vi "layout.vi"(0 "reference in":refnum<class "DQMHModuleNode.lvclass">, 1 "graph":refnum<class "Graph.lvclass">, 2 "graphics":refnum<class "Graphics.lvclass">, 3 "grid":refnum<class "Grid.lvclass">, 5 "error in (no error)":errorcluster) -> (14 "reference out":refnum<class "DQMHModuleNode.lvclass">, 19 "error out":errorcluster)   [LabVIEW 2020, in "DQMHModuleNode.lvclass"]
doc: "public void layout(Graph g, Graphics2D g2, Grid grid)"
uses:
  <resource>/Framework/Providers/Open_GDS/UML/DQMHModuleNode_class/DQMHModuleNode.lvclass
  C:/Program Files (x86)/National Instruments/LabVIEW 2020/resource/Framework/Providers/Open_GDS/UML/RectangularNode_class/RectangularNode.lvclass
  <resource>/Framework/Providers/Open_GDS/UML/Graph_class/Graph.lvclass
  <resource>/Framework/Providers/Open_GDS/UML/Graphics_class/Graphics.lvclass
  <resource>/Framework/Providers/Open_GDS/UML/Grid_class/Grid.lvclass
  <resource>/Framework/Providers/Open_GDS/UML/MultiLineString_class/MultiLineString.lvclass
  <resource>/Framework/Providers/Open_GDS/UML/RectangularNode_class/RectangularNode.lvclass
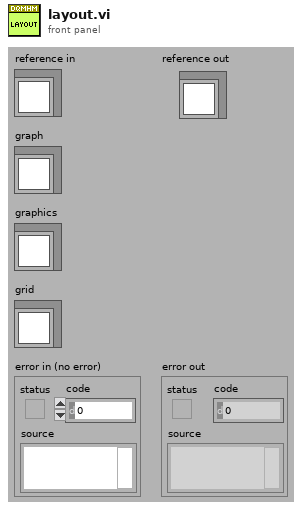
[diagram p1: front panel]
types:
  T1 = typedef "DQMHModuleNode.lvclass/ObjectAttributes.ctl" = cluster{"DescriptionHeight":dbl, "InternalDataHeight":dbl, "EventsHeight":dbl, "Name":refnum<class "MultiLineString.lvclass">, "Description":refnum<class "MultiLineString.lvclass">, "InternalData":refnum<class "MultiLineString.lvclass">, "Events":refnum<class "MultiLineString.lvclass">, "showDescription":bool, "showInternalData":bool, "showEvents":bool, "DEFAULT_ROUNDING":i32, "DEFAULT_WIDTH":i32, "DEFAULT_HEIGHT":i32, "ClassPath":path, "Template":string, "Icon":u8[][]}
  T2 = typedef "RectangularNode.lvclass/ObjectAttributes.ctl" = cluster{"bounds":T3}
  T3 = typedef "Rectangle Rectangle2D.ctl" = cluster{"x":dbl, "y":dbl, "width":dbl, "height":dbl}
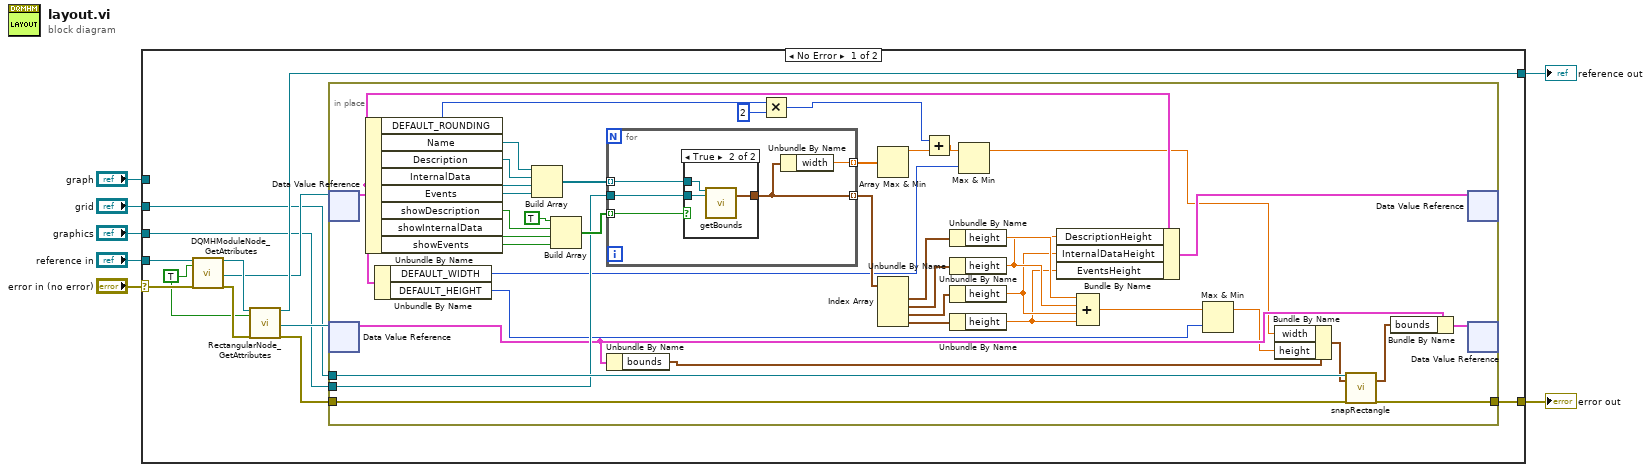
[diagram p0: block diagram]
diagram:
  n1 = case shown="No Error" "error in (no error)" {
    selector: "error in (no error)" -> [w16 w69]
    tunnel: "reference in" -> [w19 w70]
    tunnel: [w18 w69] -> w6
    tunnel: [w17 w70] -> w5
    tunnel: "graph" -> [_ _]
    tunnel: "graphics" -> [w10 _]
    tunnel: "grid" -> [w9 _]
    frame No Error {
      w8 = TRUE ("OnlyGetDvrReference(False)")
      n2 = call <resource>:"DQMHModuleNode_GetAttributes.vi"("reference in"=w19, "OnlyGetDvrReference(False)"=w8, "error in (no error)"=w16) -> ("reference out"=w15:refnum<class "DQMHModuleNode.lvclass">, "DataRef"=w13:refnum<data-value>, "error out"=w14:errorcluster)  [unwired: 13 in, 1 out]
      n3 = call <resource>:"RectangularNode_GetAttributes.vi"("reference in"=w15, "OnlyGetDvrReference(False)"=w8, "error in (no error)"=w14) -> ("reference out"=w17:refnum<class "DQMHModuleNode.lvclass">, "DataRef"=w12:refnum<data-value>, "error out"=w11:errorcluster)  [unwired: 13 in, 1 out]
      n4 = in-place {
        in-place-border: w11 -> [w25]
        in-place-border: w10 -> [w42]
        in-place-border: w9 -> [w59]
        in-place-border: [w57] -> w18
        n5 = in-place-dvr #1(w13) -> (w43:T1)  [unwired: 1 out]
        n6 = in-place-dvr #2(w12) -> (w37:T2)  [unwired: 1 out]
        n7 = Unbundle By Name(w43) -> ("DEFAULT_ROUNDING"=w21:i32, "Name"=w54:refnum<class "MultiLineString.lvclass">, "Description"=w53:refnum<class "MultiLineString.lvclass">, "InternalData"=w52:refnum<class "MultiLineString.lvclass">, "Events"=w51:refnum<class "MultiLineString.lvclass">, "showDescription"=w48:bool, "showInternalData"=w49:bool, "showEvents"=w50:bool)
        n8 = Unbundle By Name(w43) -> ("DEFAULT_WIDTH"=w29:i32, "DEFAULT_HEIGHT"=w26:i32)
        n9 = Build Array(w54, w53, w52, w51) -> (w46:refnum<class "MultiLineString.lvclass">[])
        n10 = Build Array(TRUE, w48, w49, w50) -> (w45:bool[])
        n11 = for {
          tunnel: w46 -> [w65] mode=indexing
          tunnel: w45 -> [w64] mode=indexing
          tunnel: [w62] -> w44 mode=indexing
          tunnel: w42 -> [w63]
          tunnel: [w61] -> w38 mode=indexing
          n12 = case shown="True" w64 {
            tunnel: w65 -> [_ w68]
            tunnel: [_ w67] -> w62
            tunnel: w63 -> [_ w66]
            frame False {
            }
            frame True {
              n13 = call-dynamic "getBounds.vi"("reference"=w68, "graphics"=w66) -> ("bounds"=w67:T3)  [unwired: 1 in, 16 out]
            }
          }
          n14 = Unbundle By Name(w62) -> ("width"=w61:dbl)
        }
        n15 = Unbundle By Name(w37) -> ("bounds"=w56:T3)
        n16 = Multiply(x=w21, y=2) -> (x*y=w20:i32)
        n17 = Array Max & Min(array=w38) -> (max value=w24:dbl)  [unwired: 3 out]
        n18 = Index Array(array=w44) -> (element #1=w36:T3, element #2=w41:T3, element #3=w40:T3, element #4=w39:T3)  [unwired: 4 in]
        n19 = Add(x=w20, y=w24) -> (x+y=w23:dbl)
        n20 = Unbundle By Name(w36) -> ("height"=w35:dbl)
        n21 = Unbundle By Name(w41) -> ("height"=w34:dbl)
        n22 = Unbundle By Name(w40) -> ("height"=w33:dbl)
        n23 = Unbundle By Name(w39) -> ("height"=w32:dbl)
        n24 = Max & Min(x=w23, y=w29) -> (max(x,y)=w30:dbl)  [unwired: 1 out]
        n25 = Bundle By Name(cluster=w43, "DescriptionHeight"=w34, "InternalDataHeight"=w33, "EventsHeight"=w32) -> (w60:T1)
        n26 = Compound Arithmetic op=ADD(w35, w34, w33, w32) -> (w28:dbl)
        n27 = Max & Min(x=w28, y=w26) -> (max(x,y)=w27:dbl)  [unwired: 1 out]
        n28 = Bundle By Name(cluster=w56, "width"=w30, "height"=w27) -> (w31:T3)
        n29 = call <resource>:"snapRectangle.vi"("reference"=w59, "bounds"=w31, "error in (no error)"=w25) -> ("boundsOut"=w58:T3, "error out"=w57:errorcluster)  [unwired: 15 out]
        n30 = Bundle By Name(cluster=w37, "bounds"=w58) -> (w55:T2)
        n31 = in-place-dvr #1(w60) -> ()  [unwired: 2 out]
        n32 = in-place-dvr #2(w55) -> ()  [unwired: 2 out]
      }
    }
    frame Error {
    }
  }
  "reference out" <- w5
  "error out" <- w6
